vi "PPL_Robot Main.vi"   [LabVIEW 2019]
doc: "This VI implements the framework and scheduler for your robotics program. It should not be necessary to modify the framework. You are expected to add your code to the VIs called from Robot Main - the ones located in the Team Code folder within the project."
types:
  T1 = enum32{"Invalid", "Standard", "Closed", "Hidden", "Minimized", "Maximized"}
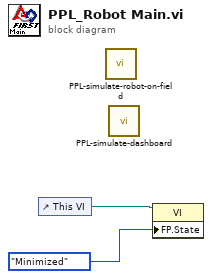
[diagram p0: block diagram]
diagram:
  n1 = control-ref of="This VI"() -> (w2:refnum<vi>)
  n2 = call "PPL-simulate-robot-on-field.vi"() -> ()  [unwired: 12 in]
  n3 = call "PPL-simulate-dashboard.vi"() -> ()  [unwired: 12 in]
  n4 = property class="VI"(reference=w2, "FP.State"=T1."Minimized" ("Front Panel Window:State")) -> ()  [unwired: 1 in, 2 out]
